vi "Route CO3000 Command.vi"(8 "error in (no error)":errorcluster caption="에러 입력(에러 없음)", 10 "문자열":string, 11 "Instrument Manager 입력":refnum<class "Instrument Manager.lvclass">) -> (0 "error out":errorcluster caption="에러 출력", 3 "Instrument Manager 출력":refnum<class "Instrument Manager.lvclass">)   [LabVIEW 2023, in "Instrument Manager.lvclass"]
uses:
  Instrument Manager.lvclass
  <vilib>/regexp/Match Regular Expression.xnode
  Instrument Manager.lvclass/Instrument Manager.ctl
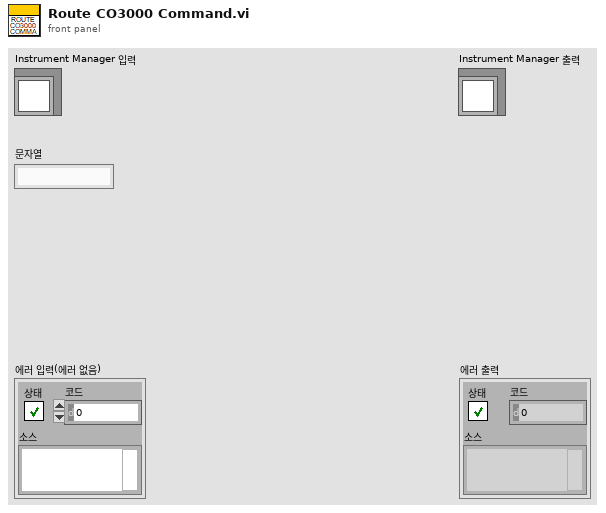
[diagram p1: front panel]
types:
  T1 = typedef "Instrument Manager.lvclass/Connect FSV Params.ctl" = cluster{"type":string, "id":string, "target":string, "command":string, "Params":cluster{"VISA Resource":string}}
  T2 = typedef "Instrument Manager.lvclass/Default Request.ctl" = cluster{"type":string, "id":string, "target":string, "command":string}
  T3 = typedef "Instrument Manager.lvclass/Change CO3000 Ant Pol Param.ctl" = cluster{"type":string, "id":string, "target":string, "command":string, "Params":cluster{"pol":string, "Mast Index":i32}}
  T4 = cluster{"Target Angle":dbl, "Turn Table Speed":i32, "Fetch Interval":i32}
  T5 = typedef "Instrument Manager.lvclass/Move TurnTable Param.ctl" = cluster{"type":string, "id":string, "target":string, "command":string, "Params":cluster{"Turn Table Info":cluster{"Target Angle":dbl, "Turn Table Speed":i32, "Fetch Interval":i32}}}
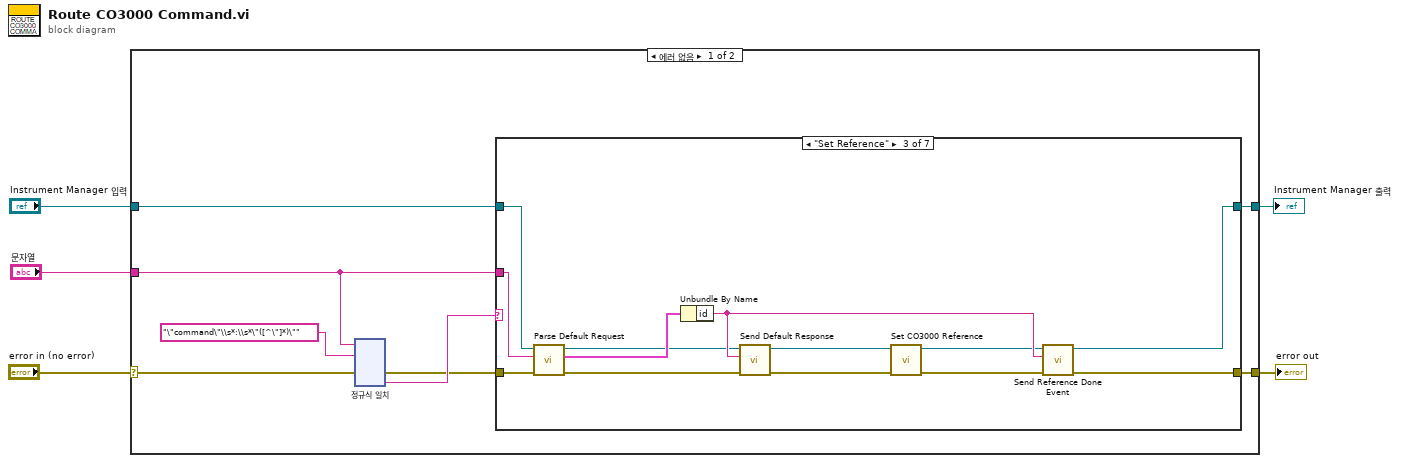
[diagram p0: block diagram]
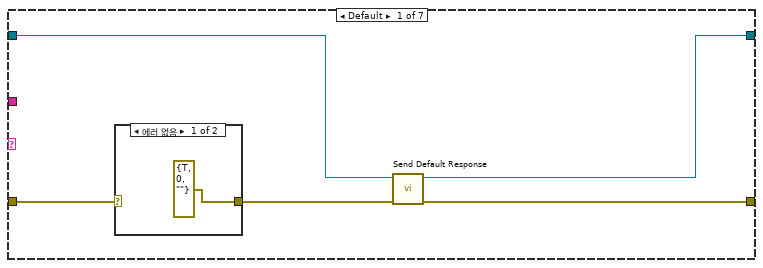
[diagram p2: hidden frame]
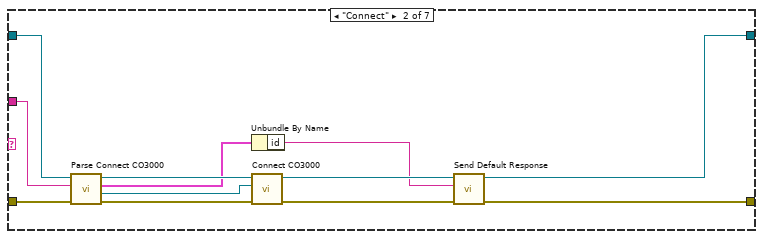
[diagram p4: hidden frame]
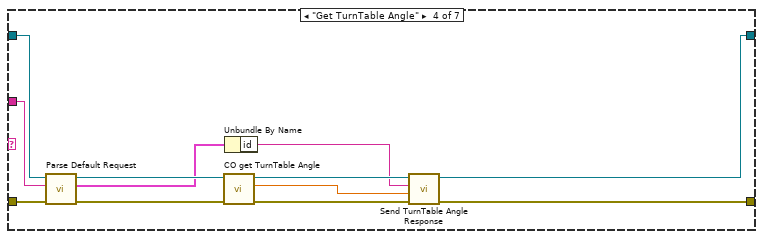
[diagram p5: hidden frame]
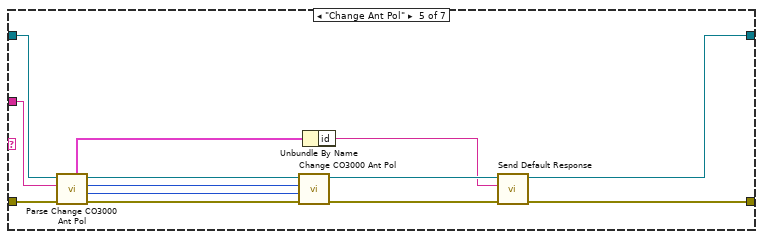
[diagram p6: hidden frame]
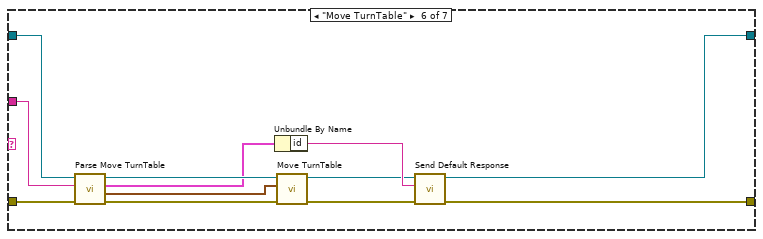
[diagram p7: hidden frame]
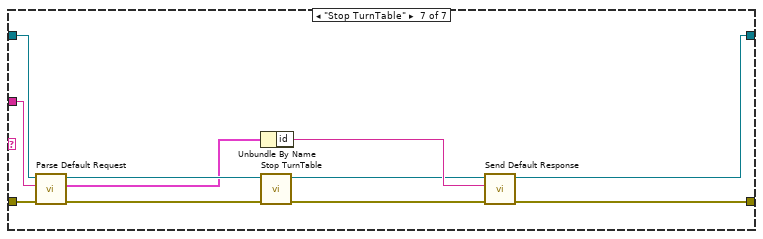
[diagram p8: hidden frame]
diagram:
  n1 = case shown="에러 없음" "error in (no error)" {
    selector: "error in (no error)" -> [w13 w214]
    tunnel: [w8 w214] -> w4
    tunnel: [w6 w213] -> w2
    tunnel: "Instrument Manager 입력" -> [w7 w213]
    tunnel: "문자열" -> [w10 _]
    frame No Error {
      n2 = xnode "정규식 일치"("입력 문자열"=w10, "정규식"="\"command\"\\s*:\\s*\"([^\"]*)\"", "에러 입력"=w13) -> ("에러 출력"=w9:errorcluster, "부분 일치 1"=w11:string)  [unwired: 3 in, 4 out]
      n3 = case shown="\"Set Reference\"" w11 {
        tunnel: w10 -> [_ w30 w44 w56 w69 w82 w92]
        tunnel: w9 -> [w17 w31 w45 w57 w70 w81 w93]
        tunnel: [w16 w21 w38 w50 w62 w73 w87] -> w8
        tunnel: w7 -> [w15 w32 w43 w55 w68 w78 w91]
        tunnel: [w14 w22 w33 w46 w61 w71 w86] -> w6
        frame Default {
          n4 = case shown="에러 없음" w17 {
            selector: w17 -> [_ w20]
            tunnel: [errorcluster {"status"=TRUE, "code"=0, "source"=""} ("error IO") w20] -> w18
            frame No Error {
            }
            frame Error {
            }
          }
          n5 = call "Send Default Response.vi"("error in (no error)"=w18, "Instrument Manager 입력"=w15) -> ("error out"=w16:errorcluster, "Instrument Manager 출력"=w14:refnum<class "Instrument Manager.lvclass">)  [unwired: 8 in]
        }
        frame "Connect" {
          n6 = call "Parse Connect CO3000.vi"("error in (no error)"=w31, "JSON string"=w30, "Instrument Manager 입력"=w32) -> ("error out"=w29:errorcluster, "VISA 리소스 이름"=w28:refnum<visa-resource-name>, "Connect FSV Param"=w24:T1, "Instrument Manager 출력"=w27:refnum<class "Instrument Manager.lvclass">)  [unwired: 5 in]
          n7 = Unbundle By Name(w24) -> ("id"=w23:string)
          n8 = call "Connect CO3000.vi"("error in (no error)"=w29, "VISA resource name"=w28, "Instrument Manager 입력"=w27) -> ("error out"=w25:errorcluster, "Instrument Manager 출력"=w26:refnum<class "Instrument Manager.lvclass">)  [unwired: 7 in]
          n9 = call "Send Default Response.vi"("error in (no error)"=w25, "id"=w23, "Instrument Manager 입력"=w26) -> ("error out"=w21:errorcluster, "Instrument Manager 출력"=w22:refnum<class "Instrument Manager.lvclass">)  [unwired: 7 in]
        }
        frame "Set Reference" {
          n10 = call "Parse Default Request.vi"("error in (no error)"=w45, "JSON string"=w44, "Instrument Manager 입력"=w43) -> ("error out"=w41:errorcluster, "Default Request"=w42:T2, "Instrument Manager 출력"=w35:refnum<class "Instrument Manager.lvclass">)  [unwired: 6 in]
          n11 = Unbundle By Name(w42) -> ("id"=w37:string)
          n12 = call "Send Default Response.vi"("error in (no error)"=w41, "id"=w37, "Instrument Manager 입력"=w35) -> ("error out"=w40:errorcluster, "Instrument Manager 출력"=w36:refnum<class "Instrument Manager.lvclass">)  [unwired: 7 in]
          n13 = call "Set CO3000 Reference.vi"("error in (no error)"=w40, "Instrument Manager 입력"=w36) -> ("error out"=w39:errorcluster, "Instrument Manager 출력"=w34:refnum<class "Instrument Manager.lvclass">)  [unwired: 8 in]
          n14 = call "Send Reference Done Event.vi"("error in (no error)"=w39, "id"=w37, "Instrument Manager 입력"=w34) -> ("error out"=w38:errorcluster, "Instrument Manager 출력"=w33:refnum<class "Instrument Manager.lvclass">)  [unwired: 7 in]
        }
        frame "Get TurnTable Angle" {
          n15 = call "Parse Default Request.vi"("error in (no error)"=w57, "JSON string"=w56, "Instrument Manager 입력"=w55) -> ("error out"=w54:errorcluster, "Default Request"=w52:T2, "Instrument Manager 출력"=w53:refnum<class "Instrument Manager.lvclass">)  [unwired: 6 in]
          n16 = call "CO get TurnTable Angle.vi"("error in (no error)"=w54, "Instrument Manager 입력"=w53) -> ("error out"=w51:errorcluster, "Current Angle"=w47:dbl, "Instrument Manager 출력"=w49:refnum<class "Instrument Manager.lvclass">)  [unwired: 7 in]
          n17 = Unbundle By Name(w52) -> ("id"=w48:string)
          n18 = call "Send TurnTable Angle Response.vi"("error in (no error)"=w51, "Current Angle"=w47, "id"=w48, "Instrument Manager 입력"=w49) -> ("error out"=w50:errorcluster, "Instrument Manager 출력"=w46:refnum<class "Instrument Manager.lvclass">)  [unwired: 6 in]
        }
        frame "Change Ant Pol" {
          n19 = call "Parse Change CO3000 Ant Pol.vi"("error in (no error)"=w70, "JSON string"=w69, "Instrument Manager 입력"=w68) -> ("error out"=w67:errorcluster, "Mast Index"=w60:i32, "Antenna Pol"=w59:enum16{"H", "V"}, "Instrument Manager 출력"=w66:refnum<class "Instrument Manager.lvclass">, "Change CO3000 Ant Pol Param"=w58:T3)  [unwired: 4 in]
          n20 = call "Change CO3000 Ant Pol.vi"("error in (no error)"=w67, "Mast Index"=w60, "Antenna Pol"=w59, "Instrument Manager 입력"=w66) -> ("error out"=w65:errorcluster, "Instrument Manager 출력"=w64:refnum<class "Instrument Manager.lvclass">)  [unwired: 6 in]
          n21 = Unbundle By Name(w58) -> ("id"=w63:string)
          n22 = call "Send Default Response.vi"("error in (no error)"=w65, "id"=w63, "Instrument Manager 입력"=w64) -> ("error out"=w62:errorcluster, "Instrument Manager 출력"=w61:refnum<class "Instrument Manager.lvclass">)  [unwired: 7 in]
        }
        frame "Move TurnTable" {
          n23 = call "Parse Move TurnTable.vi"("error in (no error)"=w81, "JSON string"=w82, "Instrument Manager 입력"=w78) -> ("error out"=w80:errorcluster, "Turn Table Info"=w79:T4, "Move TurnTable Param"=w76:T5, "Instrument Manager 출력"=w77:refnum<class "Instrument Manager.lvclass">)  [unwired: 5 in]
          n24 = Unbundle By Name(w76) -> ("id"=w75:string)
          n25 = call "Move TurnTable.vi"("error in (no error)"=w80, "Turn Table Info"=w79, "Instrument Manager 입력"=w77) -> ("error out"=w74:errorcluster, "Instrument Manager 출력"=w72:refnum<class "Instrument Manager.lvclass">)  [unwired: 7 in]
          n26 = call "Send Default Response.vi"("error in (no error)"=w74, "id"=w75, "Instrument Manager 입력"=w72) -> ("error out"=w73:errorcluster, "Instrument Manager 출력"=w71:refnum<class "Instrument Manager.lvclass">)  [unwired: 7 in]
        }
        frame "Stop TurnTable" {
          n27 = call "Parse Default Request.vi"("error in (no error)"=w93, "JSON string"=w92, "Instrument Manager 입력"=w91) -> ("error out"=w89:errorcluster, "Default Request"=w85:T2, "Instrument Manager 출력"=w90:refnum<class "Instrument Manager.lvclass">)  [unwired: 6 in]
          n28 = Unbundle By Name(w85) -> ("id"=w84:string)
          n29 = call "Stop TurnTable.vi"("error in (no error)"=w89, "Instrument Manager 입력"=w90) -> ("error out"=w88:errorcluster, "Instrument Manager 출력"=w83:refnum<class "Instrument Manager.lvclass">)  [unwired: 8 in]
          n30 = call "Send Default Response.vi"("error in (no error)"=w88, "id"=w84, "Instrument Manager 입력"=w83) -> ("error out"=w87:errorcluster, "Instrument Manager 출력"=w86:refnum<class "Instrument Manager.lvclass">)  [unwired: 7 in]
        }
      }
    }
    frame Error {
    }
  }
  "error out" <- w4
  "Instrument Manager 출력" <- w2
